vi "GLIMPSE Sequence Player.vi"() -> (8 "Sequence Range":cluster{i32, i32})   [LabVIEW 2015]
doc: "Allows the user to view and analyze a sequence of video stored as a temporary file on the disk. Also includes tools for setting areas of interest, manual tracking, automatic tracking by image fitting, etc."
uses:
  Header file data.ctl
  Seq file v 1/Offset table.ctl
  Seq file v 1/Offset.ctl
  Seq file v 1/file number.ctl
  Header2 file data.ctl
  <vilib>/vision/Image Controls.llb/IMAQ Image.ctl
  GLIMPSE Globals.vi
  <vilib>/Utility/file.llb/Write To Spreadsheet File (I64).vi
  AOI/AOI List Globals.vi
  <vilib>/Utility/NIReport.llb/NI_ReportGenerationCore.lvlib
panel:
  out "Header2 data":T1
  in  "Exit":bool
  out "Acquisition refnum array":refnum<file>[](array[refnum])
  out "file path":path
  out "Header data":T2 {"Pixel depth" items=["8 bits", "16 bits", "Float", "Complex", "RGB", "HSL"]; "time of 1st frame, \nsec since 1/1/04" format="%.2f"}
  in  "Change File":bool
  in  "Tab Control":T6(tab)
  in  "Overlay?":bool=TRUE caption="Loop?"
  in  "Frames to Step":u32=1 min=1 step=1
  in  "# Display\nWindows":i32=1 min=0 max=8 step=1
  in  "Delay between frames (msec)":i32=33 min=0 max=2147483600 step=100
  in  "Stop!":bool
  out "Time after 1st\nFrame (ms)":u32
  out "Mode":T7(ring)
  out "Time\nStamp":u32
  in  "Step Backward":bool
  in  "Step Forward":bool
  in  "Play Backward":bool
  in  "Play Forward":bool
  in  "Go to End":bool
  in  "Go to Begin":bool
  in  "Toggle beg/end":bool
  in  "Set end":bool
  in  "Set begin":bool
  in  "Loop?":bool=TRUE
  in  "Range Enabled":bool=TRUE caption="Restrict playback to range"
  in  "Frame Number":cluster{u32, u32}(slide)={10, 1} scale=1.0..13.0
  in  "Current Frame Number":u32(slide) max=13 scale=1.0..13.0
  out "Rev bkd":bool
  out "Fwd bkd":bool
  out "Stop bkgd":bool
  out "Filter":u16
  out "Field":u16
  out "Lasers":bool[](array[boolean])
  out "Flow":dbl
  out "Temp":dbl
  in  "Total FOVs":i16=4
  in  "Display FOV number":i16(slide)=1 min=1 scale=1.0..4.0
  in  "FOV Mode":T8(ring)=enum."Display all frames"
  in  "Printer":u16(ring) items=["Send To OneNote 16", "prism", "Microsoft XPS Document Writer", "Lab HP Color LaserJet M553", "Fax", "\\\\papercut\\Brandeis Ricoh Color", "\\\\papercut\\Brandeis Ricoh BW"]
  in  "Track by Curve Fitting to AOIs":bool
  in  "Print Image":bool
  in  "Save Portion of Current Frame":bool
  in  "Save Sequence":bool
  in  "Set/Modify AOIs (F8)":bool
  in  "Clear All":bool
  in  "Erase Last Row":bool
  out "Tracking Output File":path
  out "Number of Points":i16
  in  "Table":string[][](table)
  out "Pixel depth":u32(ring) items=["8 bits", "16 bits", "Float", "Complex", "RGB", "HSL"]
  out "Number of Frames":u32
  out "Frame width":i32
  out "Frame height":i32
  out "Camera":string
  out "Microscope":string
  out "Microscope software version":string
  out "Filter names":string[](array[string])
  out "Laser names":string[](array[string])
  # "These parameters are not for interactive use:"
  # "1"
  # "1"
  # "(F1)"
  # "(F2)"
  # "(F3)"
  # "(F4)"
  # "(F12)"
  # "Begin"
  # "Set"
  # "End"
  # "To add an (X, Y, T) point to table, click on image #1 with the point tool (\"+\")."
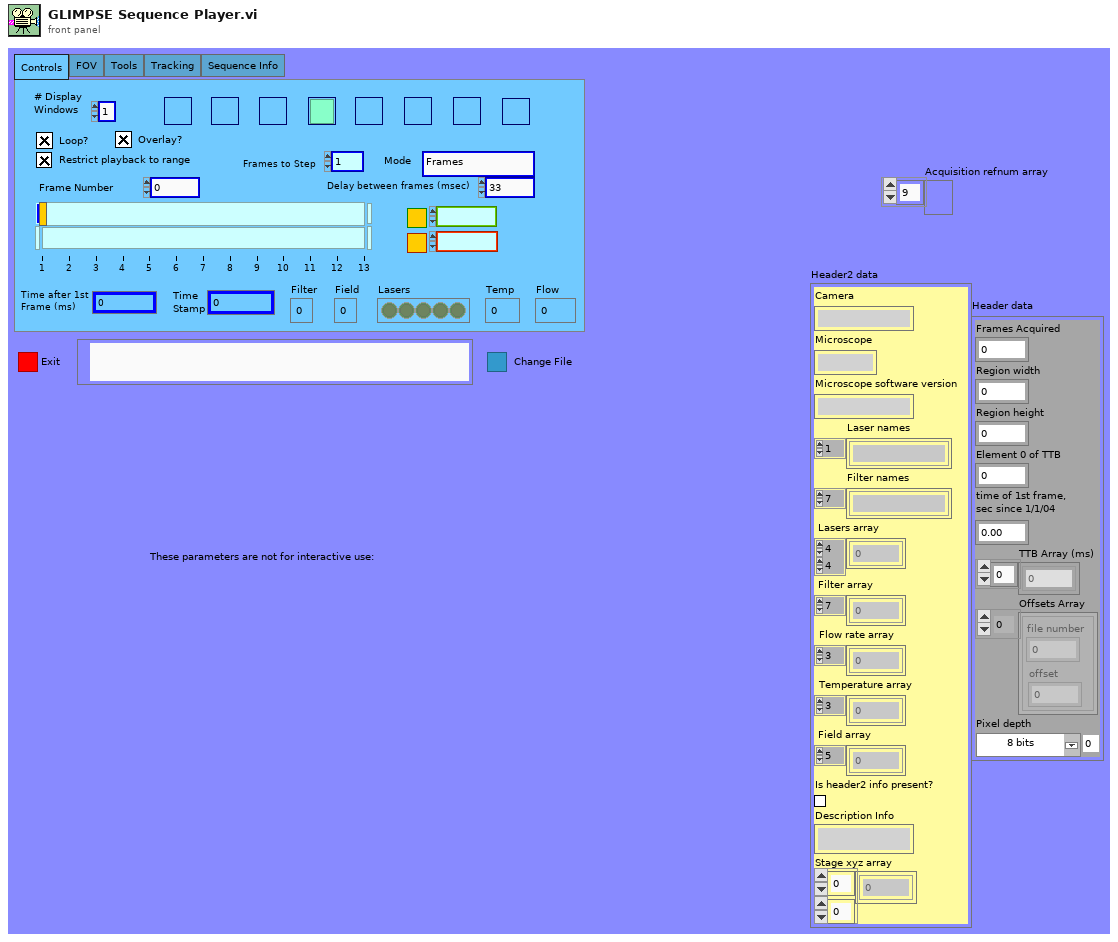
[diagram p1: front panel]
types:
  T1 = typedef "Header2 file data.ctl" = cluster{"Camera":string, "Microscope":string, "Microscope software version":string, "Laser names":string[], "Filter names":string[], "Lasers array":u16[][], "Filter array":u16[], "Flow rate array":dbl[], "Temperature array":dbl[], "Field array":u16[], "Is header2 info present?":bool, "Description Info":string, "Stage xyz array":dbl[][]}
  T2 = typedef "Header file data.ctl" = cluster{"Frames Acquired":u32, "Region width":i32, "Region height":i32, "Element 0 of TTB":u32, "time of 1st frame, \nsec since 1/1/04":dbl, "TTB Array (ms)":u32[], "Offsets Array":T3, "Pixel depth":u32}
  T3 = typedef "Offset table.ctl" = cluster{"offset":T4, "file number":T5}[]
  T4 = typedef "Offset.ctl" = i32
  T5 = typedef "file number.ctl" = u8
  T6 = enum32{"Controls", "FOV", "Tools", "Tracking", "Sequence Info"}
  T7 = enum16{"Frames", "Fields, Odd 1st", "Fields, Even 1st", "Fields, Averaged"}
  T8 = enum16{"Display one field of view", "Display all frames"}
  T9 = typedef "IMAQ Image.ctl" = refnum<image>
  T10 = enum32{"No Selection", "Point", "Line", "Rectangle", "Oval", "Polygon", "Free", "Unused1", "Zoom", "Unused2", "Broken Line", "Free Hand Line"}
  T11 = enum32{"No  event", "Click event", "Draw event", "Move event", "Size event", "Scroll event", "Activate event", "Close event", "Reserved"}[]
  T12 = cluster{"# of Frames Out (Log)":u32, "Current Frame Number":u32}
  T13 = cluster{"Left":i32, "Top":i32, "Right":i32, "Bottom":i32}
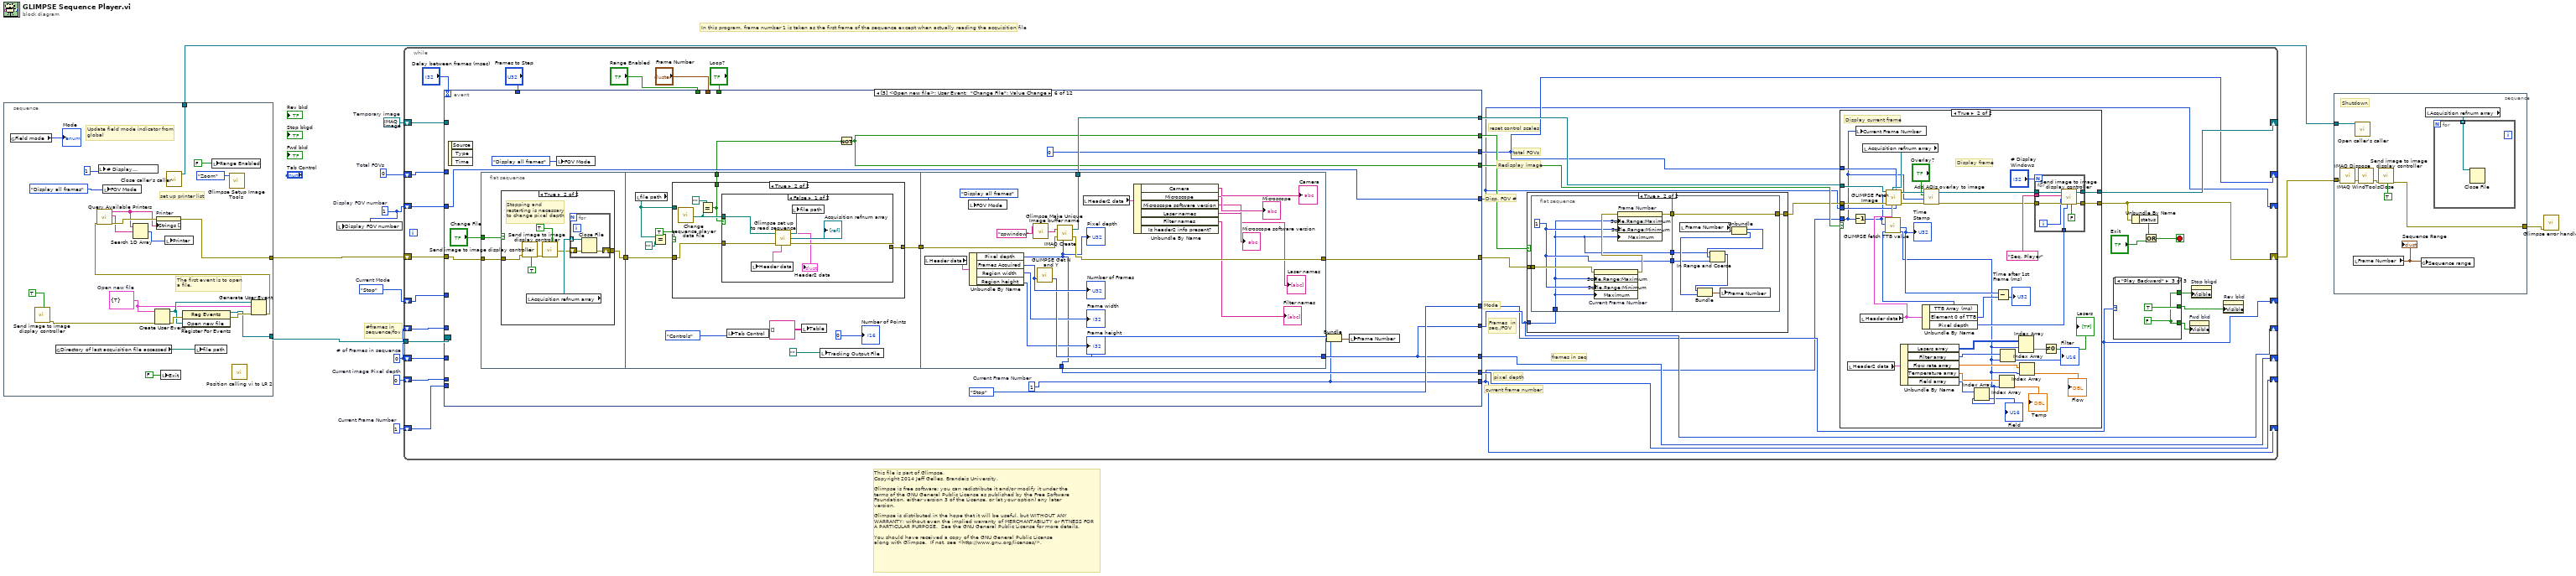
[diagram p0: block diagram]
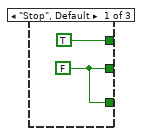
[diagram p2: hidden frame]
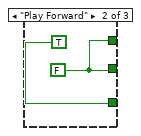
[diagram p3: hidden frame]
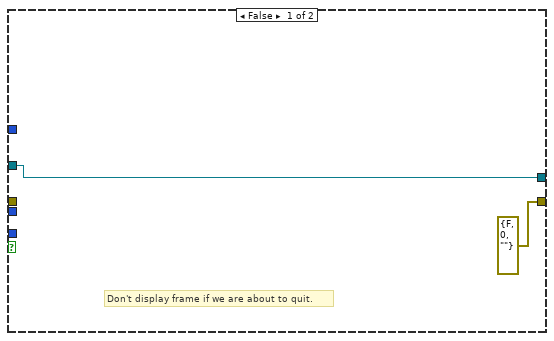
[diagram p4: hidden frame]
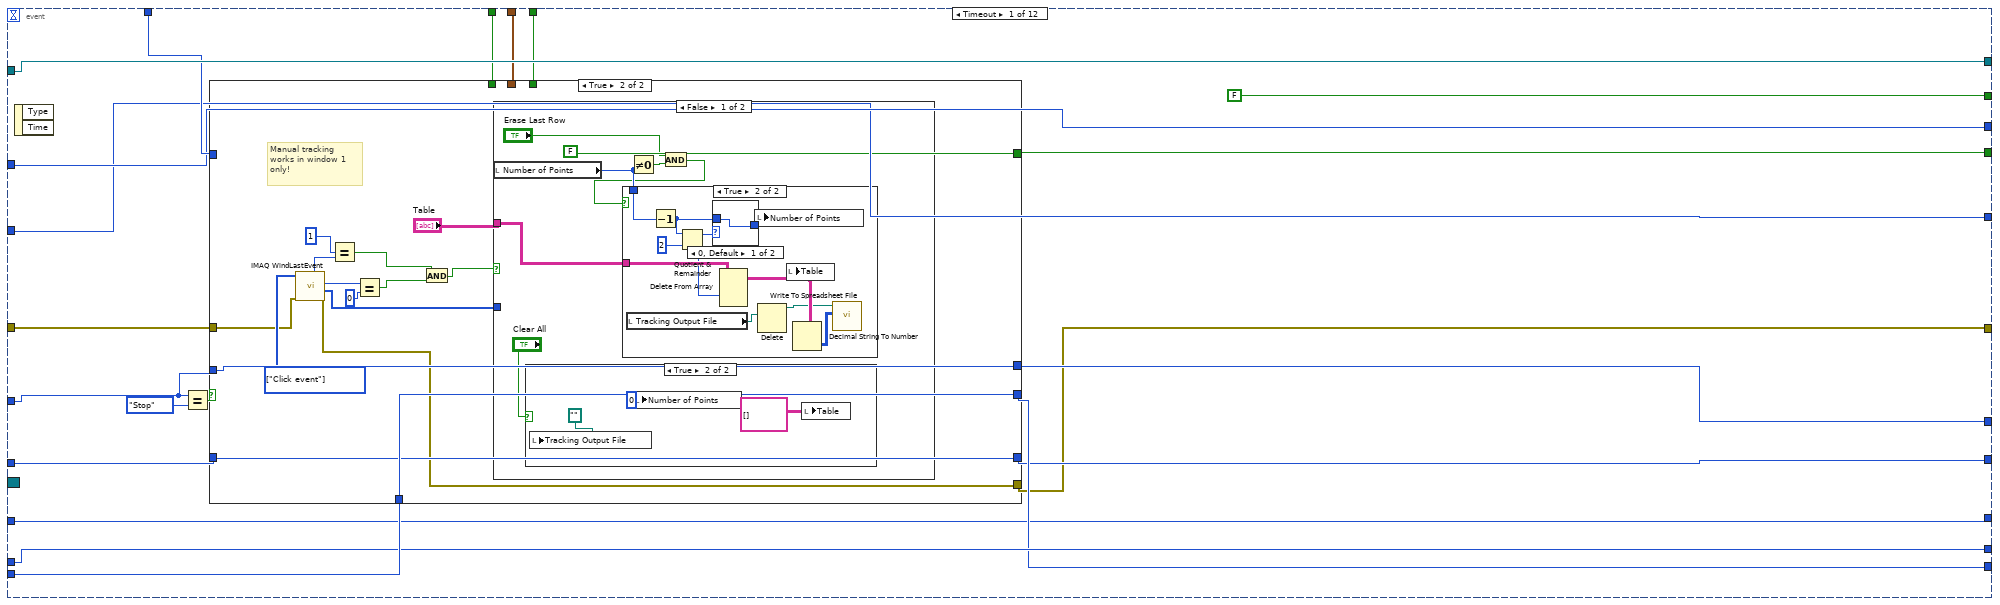
[diagram p6: hidden frame]
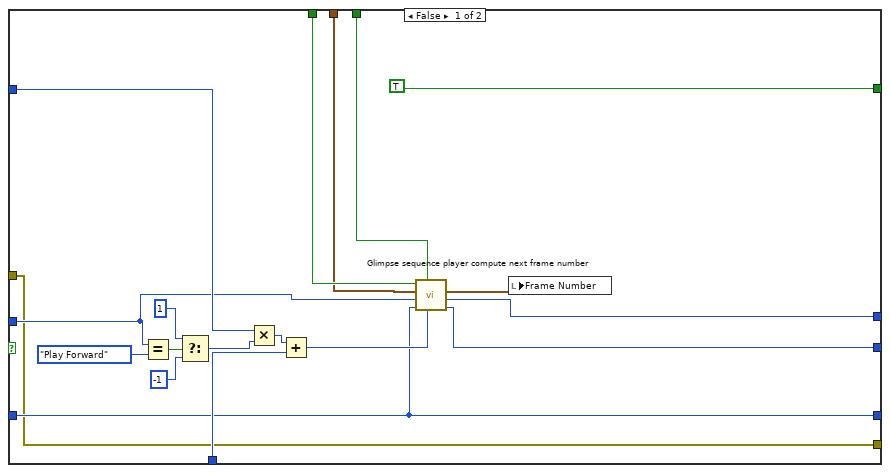
[diagram p7: hidden frame]
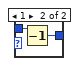
[diagram p10: hidden frame]
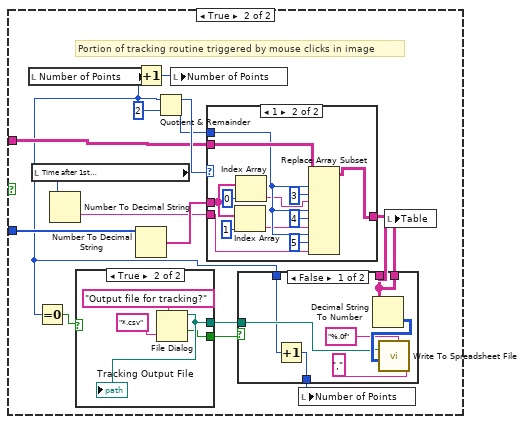
[diagram p11: hidden frame]
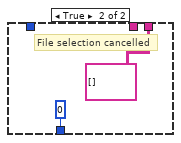
[diagram p12: hidden frame]
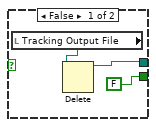
[diagram p13: hidden frame]
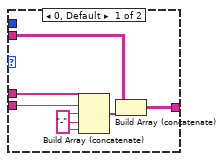
[diagram p14: hidden frame]
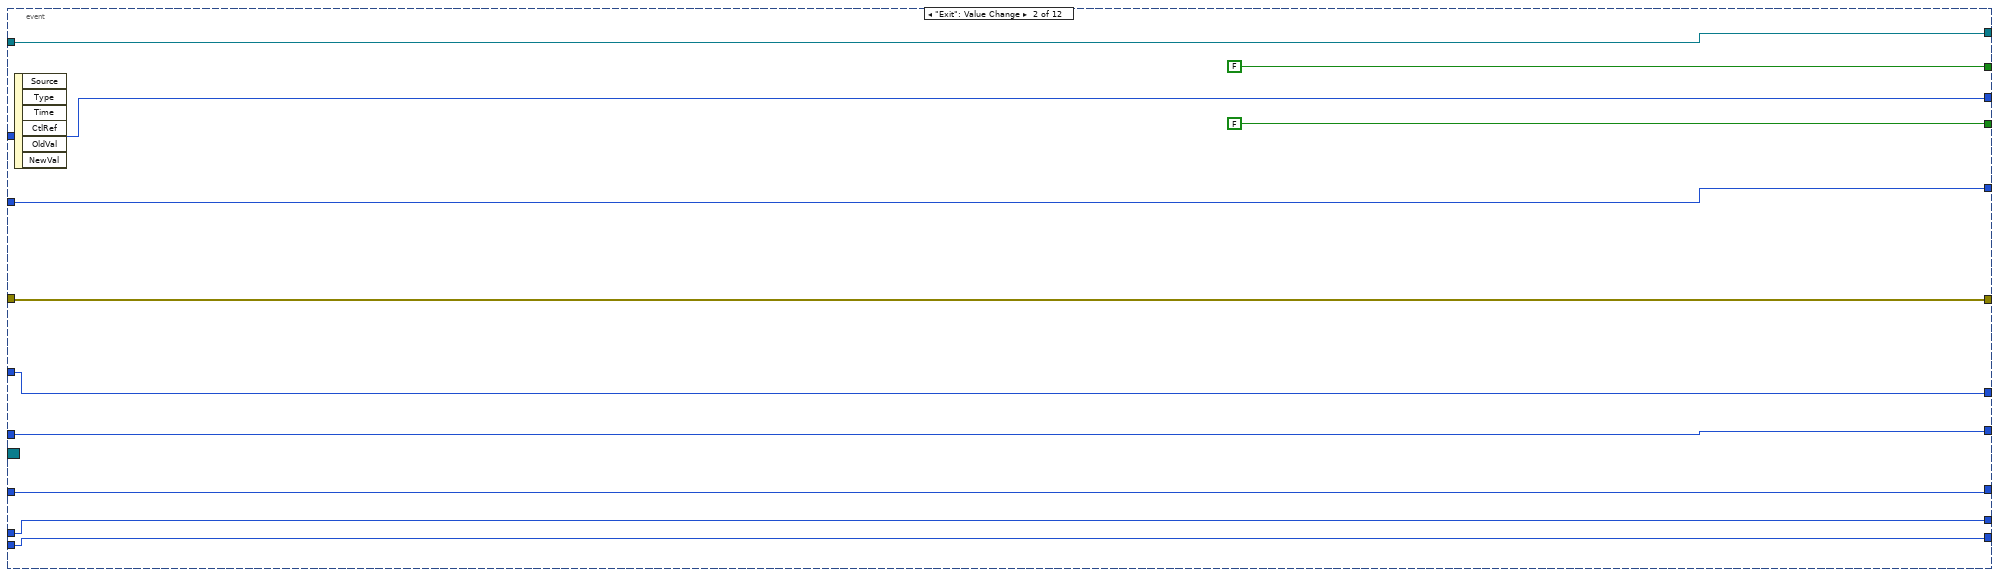
[diagram p15: hidden frame]
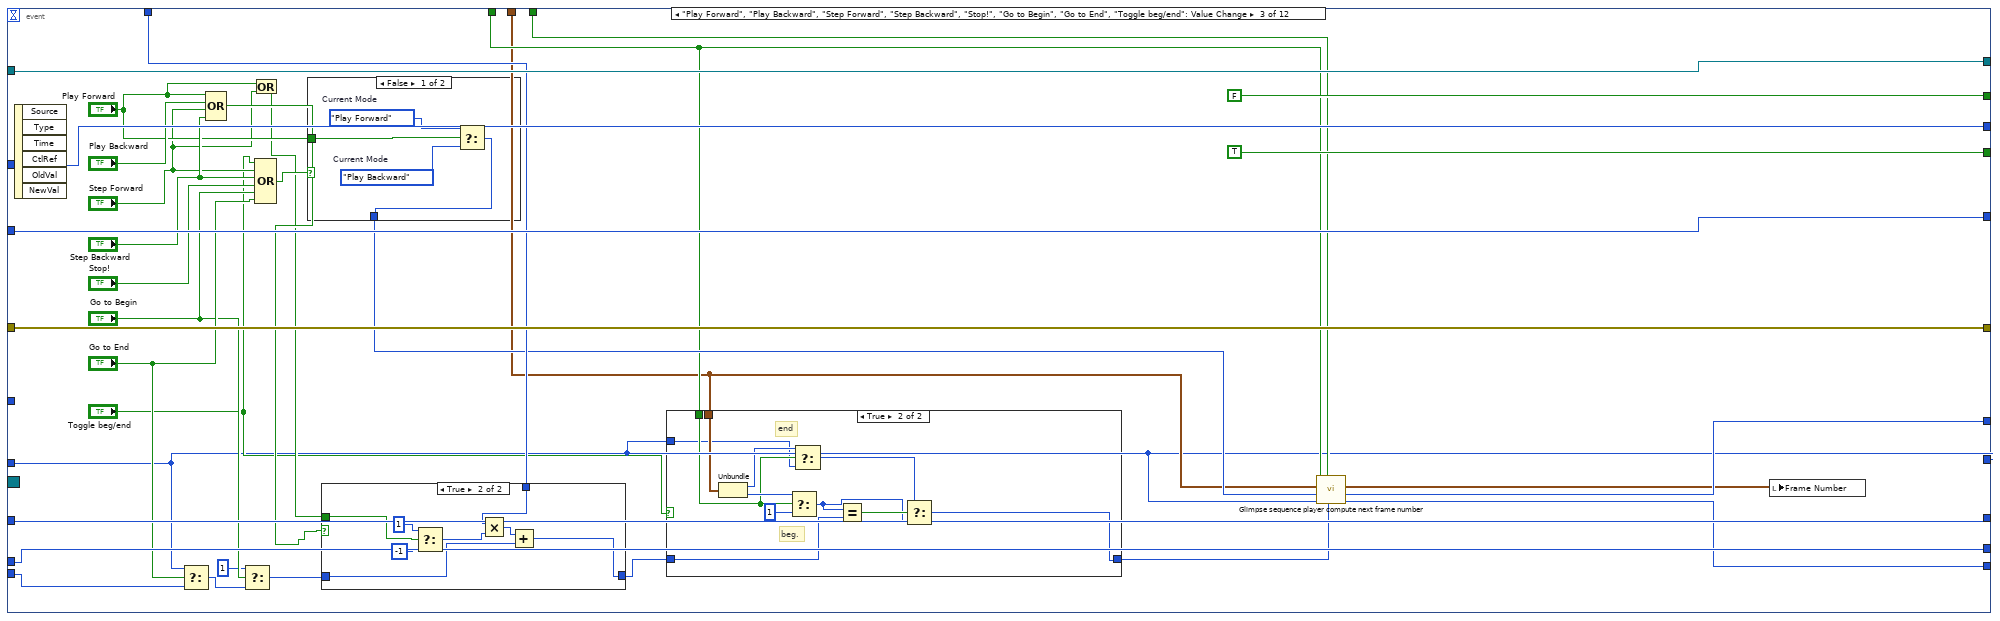
[diagram p16: hidden frame]
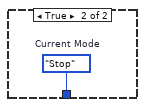
[diagram p19: hidden frame]
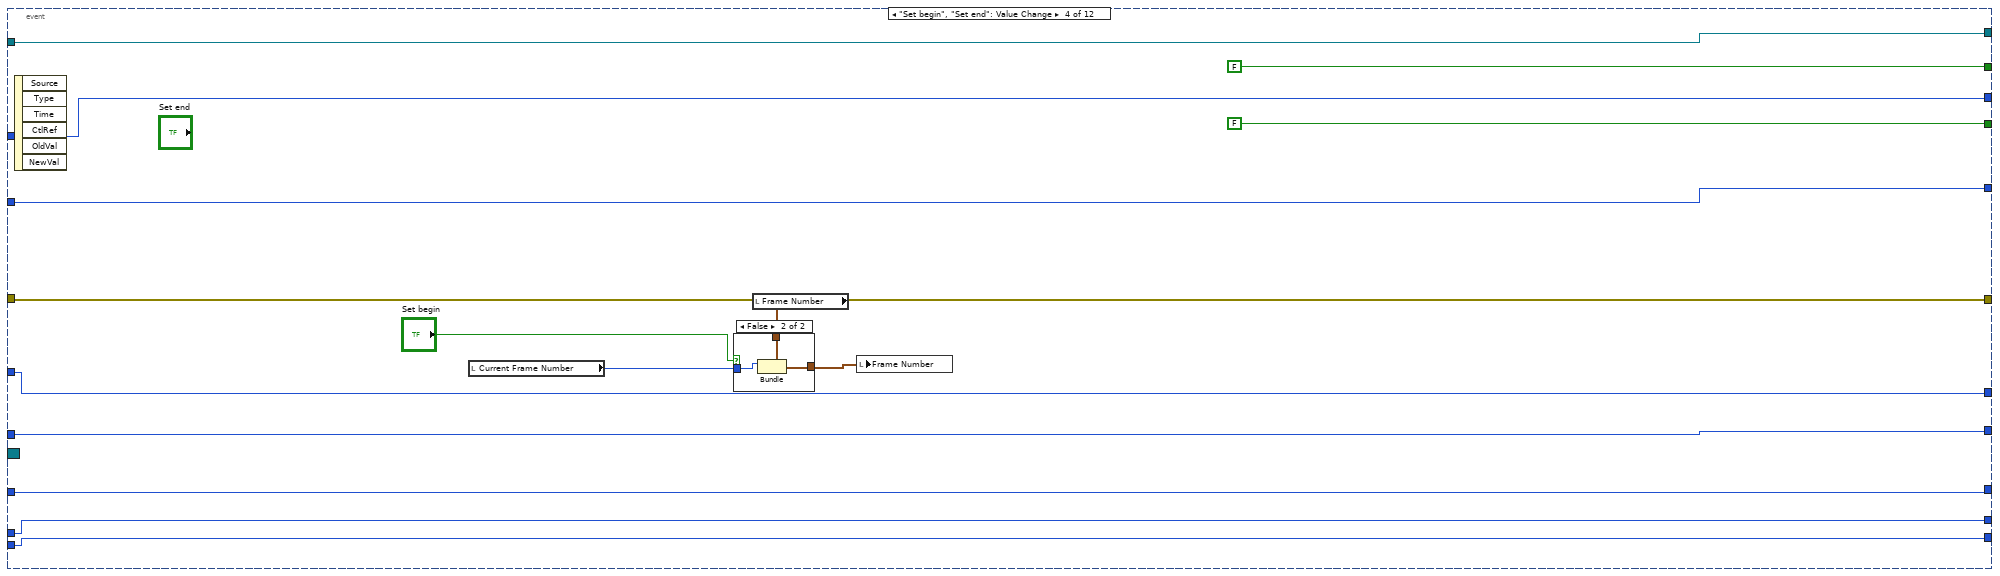
[diagram p20: hidden frame]
diagram:
  w3 = u32 0  # # of Frames in sequence
  w6 = T9 refnum  # Temporary image
  w4 = i16 1  # Display FOV number
  w7 = i16 0  # Total FOVs
  w8 = u32 0  # Current image Pixel depth
  w11 = u32 1  # Current Frame Number
  w5 = enum16{"Stop", "Play Forward", "Play Backward"}."Stop"  # Current Mode
  # "This file is part of Glimpse. \nCopyright 2014 Jeff Gelles, Brandeis University.    \n\nGlimpse is free software: you can redistribute it and/or modify it under the \nterms of the GNU General Public License as published by the Free Software \nFoundation, either version 3 of the License, or (at your option) any later \nversion.\n\nGlimpse is distributed in the hope that it will be useful, but WITHOUT ANY \nWARRANTY; without even the implied warranty of MERCHANTABILITY or FITNESS FOR \nA PARTICULAR PURPOSE.  See the GNU General Public License for more details.\n\nYou should have received a copy of the GNU General Public License\nalong with Glimpse.  If not, see <http://www.gnu.org/licenses/>."
  # "#frames in\nsequence/fov"
  # "In this program, frame number 1 is taken as the first frame of the sequence except when actually reading the acquisition file"
  n1 = stacked-sequence {
    tunnel: [w32] -> w12
    tunnel: [w21] -> w10
    tunnel: [w17] -> w9
    frame #0 {
      w14 = cluster{"dummy":bool} {"dummy"=TRUE}  # Open new file
      # "Update field mode indicator from\nglobal"
      # "The first event is to open\na file."
      # "set up printer list"
      n2 = global read "GLIMPSE Globals.vi" "Field mode"() -> (→"Mode":T7)
      n3 = call "Send image to image display controller.vi"("Start display controller?"=TRUE ("Quit display controller?")) -> ("error out"=w18:errorcluster)  [unwired: 6 in, 3 out]
      n4 = global read "GLIMPSE Globals.vi" "Directory of last acquisition file accessed"() -> (w25:path)
      n5 = local write "# Display\nWindows"(1 ("# Display\nWindows")) -> ()
      n6 = local write "FOV Mode"(T8."Display all frames" ("FOV Mode")) -> ()
      n7 = Create User Event(user event datatype=w14, error in=w18) -> (user event=w22:refnum<user-event>, error out=w24:errorcluster)
      n8 = local write "Exit"(FALSE ("Exit")) -> ()
      n9 = call "Close caller's caller.vi"() -> ("vi reference"=w32:refnum<vi>)  [unwired: 1 in, 7 out]
      n10 = register-events(error in=w24, w22) -> (reference out=w21:refnum<event-registration>, error out=w23:errorcluster)  [unwired: 1 in]
      n11 = local write "file path"(w25) -> ()
      n12 = local write "Range Enabled"(FALSE ("Exit")) -> ()
      n13 = call "Glimpse Setup Image Tools"("Default Tool"=T10."Zoom") -> ()  [unwired: 1 in, 3 out]
      n14 = call "Position calling vi to LR 2.vi"() -> ()  [unwired: 2 in, 4 out]
      n15 = Generate User Event(user event=w22, event data cluster=w14, error in=w23) -> (error out=w20:errorcluster)  [unwired: 1 in, 1 out]
      n16 = call <vilib>:"Query Available Printers.vi"("error in (no error)"=w20) -> ("error out"=w30:errorcluster, "default printer"=w29:string, "system configured printers"=w28:string[])  [unwired: 8 out]
      n17 = Search 1D Array(1D array=w28, element=w29) -> (index of element=w27:i32)  [unwired: 1 out]
      n18 = property on="Printer" class="Ring (strict)"(error in=w30, "Strings []"=w28) -> (error out=w17:errorcluster)  [unwired: 1 in, 1 out]
      n19 = local write "Printer"(w27) -> ()
    }
  }
  n20 = local write "Display FOV number"(w4) -> ()
  n21 = while {
    shift-right: [w34] -> _
    shift-left: w11 -> [w66]
    tunnel: w10 -> [w68]
    shift-right: [w43] -> w2
    shift-left: w9 -> [w67]
    shift-right: [w56] -> _
    shift-left: w6 -> [w61]
    shift-right: [w65] -> _
    shift-left: w8 -> [w64]
    shift-right: [w47] -> _
    shift-left: w7 -> [w63]
    shift-right: [w46] -> _
    shift-left: w4 -> [w62]
    shift-right: [w38] -> _
    shift-left: w5 -> [w60]
    shift-right: [w55] -> _
    shift-left: w3 -> [w59]
    shift-right: [w39] -> _
    shift-left: w3 -> [w45]
    stop <- w44 stop-if-true
    (unwired) cluster{string, u32}[] [] ("Images")
    # "pixel depth"
    # "frames in seq"
    # "Frames  in\nseq./FOV"
    # "Mode"
    # "Disp. FOV #"
    # "total FOVs"
    # "current frame number"
    # "Redisplay image"
    # "reset control scales"
    n22 = event shown="[5] <Open new file>: User Event;  \"Change File\": Value Change" {
      selector: w68 -> [_ _ _ _ _ _ _ _ _ _ _ _]
      dyn-events: _ -> [_ _ _ _ _ _ _ _ _ _ _ _]
      timeout: "Delay between frames (msec)" -> [_ _ _ _ _ _ _ _ _ _ _ _]
      tunnel: w67 -> [w141 w272 w309 w347 w366 w398 w504 w527 w551 w580 w594 w622]
      tunnel: [w158 w279 w313 w354 w372 w395 w466 w529 w550 w584 w595 w623] -> w57
      tunnel: [w140 w272 w309 w347 w366 w394 w473 w527 w538 w580 w593 w622] -> w49
      tunnel: [FALSE ("Reset control scales?") FALSE ("Reset control scales?") FALSE ("Reset control scales?") FALSE ("Reset control scales?") FALSE ("Reset control scales?") w383 w471 w531 w553 w586 TRUE ("Reset control scales?") w627] -> w58
      tunnel: w66 -> [w153 w278 w302 w353 w371 _ w463 w533 w548 w583 w601 _]
      tunnel: [w150 w278 w290 w353 w371 w386 w463 w533 w548 w583 w598 "Current Frame Number"] -> w34
      tunnel: [w151 w277 w312 w352 w370 w391 w474 w532 w547 w582 w599 w625] -> w65
      tunnel: w64 -> [w151 w277 w312 w352 w370 _ w474 w532 w547 w582 w599 w625]
      tunnel: w63 -> [w152 w269 w306 w344 w363 _ w469 w528 w543 w579 _ w618]
      tunnel: w62 -> [w143 w273 w310 w348 w367 w389 w468 w526 w540 w577 _ w619]
      tunnel: w61 -> [w158 w279 w313 w354 w372 _ w467 w529 w550 w584 w595 w623]
      tunnel: w60 -> [w155 w274 _ w349 _ _ _ _ w549 w578 w592 w621]
      tunnel: [w145 w274 w288 w349 w361 enum16{"Stop", "Play Forward", "Play Backward"}."Stop" ("Current Mode") enum16{"Stop", "Play Forward", "Play Backward"}."Stop" ("Current Mode") enum16{"Stop", "Play Forward", "Play Backward"}."Stop" ("Current Mode") w549 w578 w592 w621] -> w38
      tunnel: [w144 w276 w311 w351 w369 w387 w464 w524 w546 w581 w597 w624] -> w55
      tunnel: w59 -> [w144 w276 w311 w351 w369 _ w464 w524 w546 w581 w597 w624]
      tunnel: [w152 w269 w306 w344 w363 i16 0 ("Total FOVs") w469 w528 w543 w579 w605 w618] -> w47
      tunnel: [w143 w273 w310 w348 w367 w389 w468 w526 w540 w577 w604 w619] -> w46
      tunnel: [w142 w275 w280 w350 w368 w387 w465 w525 w545 w576 w602 w620] -> w39
      tunnel: [w156 FALSE ("Redisplay image") TRUE ("Redisplay image") FALSE ("Redisplay image") FALSE ("Redisplay image") w383 w470 w530 w552 w585 TRUE ("Redisplay image") w626] -> w50
      tunnel: w45 -> [w149 w275 w280 w350 w368 _ w465 w525 w545 w576 _ w620]
      tunnel: "Frames to Step" -> [w154 _ w294 _ _ _ _ _ _ _ _ _]
      tunnel: "Loop?" -> [w148 _ w287 _ _ _ _ _ _ _ _ _]
      tunnel: "Range Enabled" -> [w147 _ w282 _ _ _ _ _ _ _ _ _]
      tunnel: "Frame Number" -> [w146 _ w281 _ w362 _ _ _ _ _ _ _]
      event Timeout {
        n23 = event-data() -> ()  [unwired: 3 out]
        n24 = Equal?(x=w155, y=enum16{"Stop", "Play Forward", "Play Backward"}."Stop") -> (x = y?=w160:bool)
        n25 = case shown="True" w160 {
          tunnel: [TRUE ("Reset control scales?") FALSE ("Reset control scales?")] -> w156
          tunnel: w155 -> [w166 w193]
          tunnel: w154 -> [w176 _]
          tunnel: w153 -> [w171 w194]
          tunnel: [w164 w194] -> w150
          tunnel: w149 -> [w162 w192]
          tunnel: w148 -> [w169 _]
          tunnel: w147 -> [w168 _]
          tunnel: w146 -> [w167 _]
          tunnel: [w163 w193] -> w145
          tunnel: [w162 w192] -> w142
          tunnel: w141 -> [w161 w181]
          tunnel: [w161 w180] -> w140
          frame False {
            n26 = Equal?(x=w166, y=enum16{"Stop", "Play Forward", "Play Backward"}."Play Forward") -> (x = y?=w177:bool)
            n27 = Select(t=1, s=w177, f=-1) -> (s? t:f=w175:i32)
            n28 = Multiply(x=w176, y=w175) -> (x*y=w172:u32)
            n29 = Add(x=w172, y=w171) -> (x+y=w165:u32)
            n30 = call "Glimpse sequence player compute next frame number.vi"("Current Frame Number"=w165, "Loop?"=w169, "# of Frames in sequence/FOV"=w162, "Current Mode"=w166, "Range In"=w167, "Range Enabled"=w168) -> ("Current Frame Number Out"=w164:u32, "Current Mode Out"=w163:enum16{"Stop", "Play Forward", "Play Backward"}, "Range Out"=w170:cluster{"Max":u32, "Min":u32})  [unwired: 1 out]
            n31 = local write "Frame Number"(w170) -> ()
          }
          frame True {
            w190 = T11 [enum."Click event"] items=["No  event", "Click event", "Draw event", "Move event", "Size event", "Scroll event", "Activate event", "Close event", "Reserved"] ("Events list (all)")
            # "Manual tracking \nworks in window 1\nonly!"
            n32 = call "IMAQ WindLastEvent"("error in (no error)"=w181, "Events list (all)"=w190) -> ("error out"=w180:errorcluster, "Coordinates"=w184:i32[], "Tool"=w189:i32, "Window Number (0...15)"=w191:i32)  [unwired: 6 out]
            n33 = Equal?(x=1 ("Window Number (0...15)"), y=w191) -> (x = y?=w186:bool)
            n34 = Equal?(x=w189, y=0) -> (x = y?=w187:bool)
            n35 = And(x=w186, y=w187) -> (x .and. y?=w185:bool)
            n36 = case shown="False" w185 {
              tunnel: w184 -> [_ w230]
              tunnel: "Table" -> [w200 w224]
              frame False {
                n37 = local read "Number of Points"() -> (w199:i16)
                n38 = case shown="True" "Clear All" {
                  frame False {
                  }
                  frame True {
                    n39 = local write "Tracking Output File"(path "") -> ()
                    n40 = local write "Number of Points"(i16 0 ("Number of Points")) -> ()
                    n41 = local write "Table"(string[][] []) -> ()
                  }
                }
                n42 = Not Equal To 0?(x=w199) -> (x != 0?=w198:bool)
                n43 = And(x="Erase Last Row", y=w198) -> (x .and. y?=w197:bool)
                n44 = case shown="True" w197 {
                  tunnel: w200 -> [_ w211]
                  tunnel: w199 -> [_ w206]
                  frame False {
                  }
                  frame True {
                    n45 = local read "Tracking Output File"() -> (w205:path)
                    n46 = Decrement(x=w206) -> (x-1=w214:i16)
                    n47 = Quotient & Remainder(x=w214, y=i16 2) -> (x-y*floor(x/y)=w212:i16, floor(x/y)=w210:i16)
                    n48 = case shown="0, Default" w212 {
                      tunnel: w214 -> [w216 w218]
                      tunnel: [w216 w217] -> w213
                      frame 0, Default {
                      }
                      frame 1 {
                        n49 = Decrement(x=w218) -> (x-1=w217:i16)
                      }
                    }
                    n50 = Delete From Array(array=w211, index (row)=w210) -> (array with subset deleted=w209:string[][])  [unwired: 2 in, 1 out]
                    n51 = local write "Number of Points"(w213) -> ()
                    n52 = Delete(path (use dialog)=w205) -> (deleted path=w208:path)  [unwired: 1 in, 5 out]
                    n53 = local write "Table"(w209) -> ()
                    n54 = Decimal String To Number(string=w209) -> (number=w207:i32[][])  [unwired: 3 out]
                    n55 = call-poly <vilib>:"Write To Spreadsheet File.vi"("2D data"=w207, "file path (dialog if empty)"=w208) -> ()  [unwired: 4 in, 3 out]
                  }
                }
              }
              frame True {
                # "Portion of tracking routine triggered by mouse clicks in image"
                n56 = local read "Number of Points"() -> (w221:i16)
                n57 = local read "Time after 1st\nFrame (ms)"() -> (w231:u32)
                n58 = Equal To 0?(x=w221) -> (x = 0?=w226:bool)
                n59 = Number To Decimal String(number=w231) -> (decimal integer string=w228:string)  [unwired: 1 out]
                n60 = case shown="True" w226 {
                  tunnel: [w245 w248] -> w222
                  tunnel: [FALSE ("cancelled") w247] -> w223
                  frame False {
                    n61 = local read "Tracking Output File"() -> (w246:path)
                    n62 = Delete(path (use dialog)=w246) -> (deleted path=w245:path)  [unwired: 1 in, 5 out]
                  }
                  frame True {
                    n63 = File Dialog(6:"*.csv" ("pattern"), 7:"Output file for tracking?" ("prompt")) -> (1:w247:bool, 3:w248:path)  [unwired: 1 in, 6 out]
                    "Tracking Output File" <- w248
                  }
                }
                n64 = Increment(x=w221) -> (x+1=w233:i16)
                n65 = Number To Decimal String(number=w230) -> (decimal integer string=w229:string[])  [unwired: 1 in]
                n66 = Quotient & Remainder(x=w221, y=i16 2) -> (x-y*floor(x/y)=w232:i16, floor(x/y)=w227:i16)
                n67 = local write "Number of Points"(w233) -> ()
                n68 = case shown="1" w232 {
                  tunnel: w224 -> [w256 w268]
                  tunnel: [w253 w267] -> w225
                  tunnel: w229 -> [w252 w261]
                  tunnel: w228 -> [w251 w262]
                  tunnel: w227 -> [_ w263]
                  frame 0, Default {
                    w254 = "-"
                    n69 = Build Array (concatenate)(w252, w251, w254, w254, w254) -> (w255:string[])
                    n70 = Build Array (concatenate)(w256, w255) -> (w253:string[][])
                  }
                  frame 1 {
                    n71 = Index Array(array=w261, index=1 ("Index")) -> (element=w257:string)
                    n72 = Index Array(array=w261, index=0 ("Index")) -> (element=w258:string)
                    n73 = Replace Array Subset(array=w268, new element #1=w258, index (row) #1=w263, index (col) #1=3 ("Disabled Index (col)"), new element #2=w257, index (row) #2=w263, index (col) #2=4 ("Index (col)"), new element #3=w262, index (row) #3=w263, index (col) #3=5 ("Index (col)")) -> (w267:string[][])
                  }
                }
                n74 = case shown="False" w223 {
                  tunnel: w225 -> [w237 _]
                  tunnel: w222 -> [w240 _]
                  tunnel: w221 -> [w239 _]
                  tunnel: [w238 i16 0] -> w220
                  tunnel: [w237 string[][] []] -> w219
                  frame False {
                    n75 = Increment(x=w239) -> (x+1=w238:i16)
                    n76 = Decimal String To Number(string=w237) -> (number=w241:i32[][])  [unwired: 3 out]
                    n77 = call-poly <vilib>:"Write To Spreadsheet File.vi"("delimiter (\\t)"="," ("delimiter (Tab)"), "format (%d)"="%.0f" ("format (%.3f)"), "2D data"=w241, "file path (dialog if empty)"=w240) -> ()  [unwired: 3 in, 2 out]
                  }
                  frame True {
                    # "File selection cancelled"
                  }
                }
                n78 = local write "Number of Points"(w220) -> ()
                n79 = local write "Table"(w219) -> ()
              }
            }
          }
        }
      }
      event "Exit": Value Change {
        n80 = event-data() -> ()  [unwired: 7 out]
      }
      event "Play Forward", "Play Backward", "Step Forward", "Step Backward", "Stop!", "Go to Begin", "Go to End", "Toggle beg/end": Value Change {
        n81 = event-data() -> ()  [unwired: 7 out]
        n82 = Select(t=w280, s="Go to End", f=w302) -> (s? t:f=w300:u32)
        n83 = Compound Arithmetic op=OR("Play Forward", "Play Backward", "Step Forward", "Step Backward") -> (w296:bool)
        n84 = Select(t=u32 1, s="Go to Begin", f=w300) -> (s? t:f=w295:u32)
        n85 = Or(x="Play Forward", y="Step Forward") -> (x .or. y?=w291:bool)
        n86 = Compound Arithmetic op=OR("Toggle beg/end", "Step Forward", "Step Backward", "Stop!", "Go to Begin", "Go to End") -> (w304:bool)
        n87 = case shown="False" w304 {
          tunnel: [w335 w339] -> w289
          tunnel: "Play Forward" -> [w338 _]
          frame False {
            w336 = enum16{"Stop", "Play Forward", "Play Backward"}."Play Backward"  # Current Mode
            w337 = enum16{"Stop", "Play Forward", "Play Backward"}."Play Forward"  # Current Mode
            n88 = Select(t=w337, s=w338, f=w336) -> (s? t:f=w335:enum16{"Stop", "Play Forward", "Play Backward"})
          }
          frame True {
            w339 = enum16{"Stop", "Play Forward", "Play Backward"}."Stop"  # Current Mode
          }
        }
        n89 = case shown="True" w296 {
          tunnel: w295 -> [w326 w329]
          tunnel: [w326 w328] -> w284
          tunnel: w294 -> [_ w330]
          tunnel: w291 -> [_ w327]
          frame False {
          }
          frame True {
            n90 = Select(t=1, s=w327, f=-1) -> (s? t:f=w332:i32)
            n91 = Multiply(x=w330, y=w332) -> (x*y=w334:u32)
            n92 = Add(x=w334, y=w329) -> (x+y=w328:u32)
          }
        }
        n93 = case shown="True" "Toggle beg/end" {
          tunnel: w284 -> [w314 w324]
          tunnel: [w314 w315] -> w283
          tunnel: w282 -> [_ w319]
          tunnel: w281 -> [_ w322]
          tunnel: w280 -> [_ w317]
          frame False {
          }
          frame True {
            # "end"
            # "beg."
            n94 = Unbundle(w322) -> (w318:u32, w321:u32)
            n95 = Select(t=w321, s=w319, f=u32 1) -> (s? t:f=w320:u32)
            n96 = Select(t=w318, s=w319, f=w317) -> (s? t:f=w316:u32)
            n97 = Equal?(x=w320, y=w324) -> (x = y?=w323:bool)
            n98 = Select(t=w316, s=w323, f=w320) -> (s? t:f=w315:u32)
          }
        }
        n99 = call "Glimpse sequence player compute next frame number.vi"("Current Frame Number"=w283, "Loop?"=w287, "# of Frames in sequence/FOV"=w280, "Current Mode"=w289, "Range In"=w281, "Range Enabled"=w282) -> ("Current Frame Number Out"=w290:u32, "Current Mode Out"=w288:enum16{"Stop", "Play Forward", "Play Backward"}, "Range Out"=w286:cluster{"Max":u32, "Min":u32})  [unwired: 1 out]
        n100 = local write "Frame Number"(w286) -> ()
      }
      event "Set begin", "Set end": Value Change {
        n101 = event-data() -> ()  [unwired: 7 out]
        n102 = local read "Current Frame Number"() -> (w342:u32)
        n103 = local read "Frame Number"() -> (w341:cluster{u32, u32})
        n104 = case shown="False" "Set begin" {
          tunnel: [w357 w360] -> w343
          tunnel: w342 -> [w356 w358]
          tunnel: w341 -> [w355 w359]
          frame True {
            n105 = Bundle(cluster=w355, w356) -> (w357:cluster{u32, u32})  [unwired: 1 out]
          }
          frame False {
            n106 = Bundle(cluster=w359, w358) -> (w360:cluster{u32, u32})  [unwired: 1 out]
          }
        }
        n107 = local write "Frame Number"(w343) -> ()
      }
      event "Track by Curve Fitting to AOIs": Value Change {
        n108 = event-data() -> ()  [unwired: 7 out]
        n109 = flat-sequence {
          tunnel: [enum16{"Stop", "Play Forward", "Play Backward"}."Stop" ("Current Mode")] -> w361
          tunnel: w362 -> [w373]
          frame #0 {
            n110 = global read "GLIMPSE Globals.vi" "Current window Black/White Levels"() -> (w374:cluster{ext, ext})
            n111 = local read "Acquisition refnum array"() -> (w380:refnum<file>[])
            n112 = local read "Header data"() -> (w375:T2)
            n113 = Unbundle(w373) -> (w379:u32, w378:u32)
            n114 = Unbundle(w374) -> (w377:ext, w376:ext)
            n115 = call "fit aois.vi"("End frame"=w379, "White level"=w376, "Header Info"=w375, "Start frame"=w378, "Black level"=w377, "Acquisition refnum array"=w380) -> ()  [unwired: 5 out]
          }
          frame #1 {
            n116 = call "IMAQ WindToolsShow"() -> ("error out"=w382:errorcluster)  [unwired: 3 in, 3 out]
            n117 = call <vilib>:"Simple Error Handler.vi"("error in (no error)"=w382) -> ()  [unwired: 1 in, 8 out]
          }
        }
      }
      event User Event; "Change File": Value Change {
        w386 = u32 1  # Current Frame Number
        n118 = event-data() -> ()  [unwired: 4 out]
        n119 = flat-sequence {
          tunnel: w398 -> [w401]
          tunnel: [w400] -> w397
          tunnel: "Change File" -> [w399]
          tunnel: w397 -> [w420]
          tunnel: [w415] -> w396
          tunnel: [w413] -> w384
          tunnel: w396 -> [w459]
          tunnel: [w458] -> w395
          tunnel: [w457] -> w394
          tunnel: [w451] -> w391
          tunnel: [w455] -> w387
          frame #0 {
            n120 = case shown="True" w399 {
              tunnel: w401 -> [w402 w407]
              tunnel: [w402 w406] -> w400
              frame False {
              }
              frame True {
                # "Stopping and \nrestarting is necessary\nto change pixel depth"
                n121 = call "Send image to image display controller.vi"("error in"=w407, "Quit display controller?"=TRUE) -> ("error out"=w403:errorcluster)  [unwired: 5 in, 3 out]
                n122 = local read "Acquisition refnum array"() -> (w409:refnum<file>[])
                n123 = call "Send image to image display controller.vi"("error in"=w403, "Start display controller?"=TRUE ("Quit display controller?")) -> ("error out"=w408:errorcluster)  [unwired: 5 in, 3 out]
                n124 = for {
                  tunnel: w409 -> [w412] mode=indexing
                  shift-right: [w410] -> w406
                  shift-left: w408 -> [w411]
                  n125 = Close File(refnum=w412, error in=w411) -> (error out=w410:errorcluster)  [unwired: 1 out]
                }
              }
            }
          }
          frame #1 {
            n126 = local read "file path"() -> (w422:path)
            n127 = Equal?(x=w422, y=path "") -> ()  [unwired: 1 out]
            n128 = case shown="True" TRUE {
              tunnel: w422 -> [w430 _]
              tunnel: w420 -> [w426 w433]
              tunnel: [w425 w432] -> w415
              tunnel: [FALSE w431] -> w413
              frame False {
                # "automatically open last file accessed"
                n129 = call "Glimpse set up to read sequence.vi"("acquisition directory path"=w430, "error in"=w426) -> ("Header2 file data out"=w423:T1, "Header file data out"=→"Header data":T2, "acquisition directory path out"=→"file path":path, "Acquisition refnum array"=w428:refnum<file>[], "error out"=w425:errorcluster)  [unwired: 1 out]
                n130 = local write "Acquisition refnum array"(w428) -> ()
                n131 = local write "Header2 data"(w423) -> ()
              }
              frame True {
                n132 = call "Change sequence player data file.vi"() -> ("File path out"=w435:path)  [unwired: 1 in, 4 out]
                n133 = Equal?(x=path "", y=w435) -> (x = y?=w431:bool)
                n134 = case shown="False" w431 {
                  tunnel: w435 -> [w442 _]
                  tunnel: w433 -> [w438 w444]
                  tunnel: [w437 w444] -> w432
                  frame False {
                    n135 = call "Glimpse set up to read sequence.vi"("acquisition directory path"=w442, "error in"=w438) -> ("Header2 file data out"=→"Header2 data":T1, "Header file data out"=w439:T2, "acquisition directory path out"=w441:path, "Acquisition refnum array"=→"Acquisition refnum array":refnum<file>[], "error out"=w437:errorcluster)  [unwired: 1 out]
                    n136 = local write "Header data"(w439) -> ()
                    n137 = local write "file path"(w441) -> ()
                  }
                  frame True {
                    n138 = local write "Exit"(TRUE ("Exit")) -> ()
                  }
                }
              }
            }
            n139 = local write "Tab Control"(enum32{"Controls", "FOV", "Tools", "Tracking"}."Controls" ("Tab Control")) -> ()
            n140 = local write "Table"(string[][] []) -> ()
            n141 = local write "Tracking Output File"(path "") -> ()
            "Number of Points" <- i16 0 ("Number of Points")
          }
          frame #2 {
            n142 = local read "Header data"() -> (w462:T2)
            n143 = local write "FOV Mode"(T8."Display all frames" ("FOV Mode")) -> ()
            n144 = Unbundle By Name(w462) -> ("Pixel depth"=w451:u32, "Frames Acquired"=w456:u32, "Region width"=→"Frame width":i32, "Region height"=→"Frame height":i32)
            "Number of Frames" <- w456
            "Pixel depth" <- w451
            n145 = call "Glimpse Make Unique Image buffer name.vi"("Buffer  base name"="spwindow" ("Image Name")) -> ("Image Name"=w461:string)  [unwired: 1 out]
            n146 = call "GLIMPSE Get N and Y.vi"("# of Frames In (Phys)"=w456) -> ("# of Frames Out (Log)"=w455:u32)  [unwired: 2 in, 4 out]
            n147 = call "IMAQ Create"("Image Name"=w461, "Image Type"=w451, "error in (no error)"=w459) -> ("New Image"=w458:T9, "error out"=w457:errorcluster)  [unwired: 1 in, 1 out]
            n148 = local read "Header2 data"() -> (w450:T1)
            n149 = Unbundle By Name(w450) -> ("Camera"=→"Camera":string, "Microscope"=→"Microscope":string, "Microscope software version"=→"Microscope software version":string, "Laser names"=→"Laser names":string[], "Filter names"=→"Filter names":string[])  [unwired: 1 out]
          }
        }
        n150 = local write "FOV Mode"(T8."Display all frames" ("FOV Mode")) -> ()
        n151 = Not(x=w384) -> (.not. x?=w383:bool)
        n152 = Bundle("# of Frames Out (Log)"=w387, "Current Frame Number"=w386) -> (w388:T12)  [unwired: 1 out]
        n153 = local write "Frame Number"(w388) -> ()
      }
      event "Set/Modify AOIs (F8)": Value Change {
        w470 = TRUE  # Redisplay image
        w471 = FALSE  # Reset control scales?
        n154 = event-data() -> ()  [unwired: 7 out]
        n155 = call "IMAQ Create"("Image Name"="Field1", "Image Type"=w474, "error in (no error)"=w504) -> ("New Image"=w508:T9, "error out"=w501:errorcluster)  [unwired: 1 in, 1 out]
        n156 = call "IMAQ Create"("Image Name"="Field2", "Image Type"=w474, "error in (no error)"=w501) -> ("New Image"=w507:T9, "error out"=w480:errorcluster)  [unwired: 1 in, 1 out]
        n157 = local read "Header data"() -> (w481:T2)
        n158 = local read "Frame Number"() -> (w498:cluster{u32, u32})
        n159 = global read "GLIMPSE Globals.vi" "Current window Black/White Levels"() -> (w492:cluster{ext, ext})
        n160 = Unbundle(w498) -> (w500:u32, w499:u32)
        n161 = Decrement(x=w500) -> (x-1=w497:u32)
        n162 = Decrement(x=w499) -> (x-1=w496:u32)
        n163 = local read "Acquisition refnum array"() -> (w495:refnum<file>[])
        n164 = call "GLIMPSE Fetch Image.vi"("Display FOV number"=w468, "Total FOVs"=w469, "Header file data"=w481, "Acqisition files refnums"=w495, "error in"=w480, "Logical Frame Number\n(starting with zero)"=w497, "Image In"=w508) -> ("error out"=w479:errorcluster, "Image Out"=w506:T9)  [unwired: 3 out]
        n165 = call "GLIMPSE Fetch Image.vi"("Display FOV number"=w468, "Total FOVs"=w469, "Header file data"=w481, "Acqisition files refnums"=w495, "error in"=w479, "Logical Frame Number\n(starting with zero)"=w496, "Image In"=w507) -> ("error out"=w478:errorcluster, "Image Out"=w505:T9)  [unwired: 3 out]
        n166 = Unbundle(w492) -> (w494:ext, w493:ext)
        n167 = call "Multiple AOIs.vi"("White level"=w493, "Black level"=w494, "First (or only) image (red)"=w506, "error in"=w478, "Second image (green)"=w505, "Image Type"=w474) -> ("error out"=w477:errorcluster)  [unwired: 5 out]
        n168 = call "IMAQ WindToolsShow"("error in (no error)"=w477) -> ("error out"=w490:errorcluster)  [unwired: 2 in, 3 out]
        n169 = local write "Tab Control"(enum32{"Controls", "FOV", "Tools", "Tracking"}."Controls" ("Tab Control")) -> ()
        n170 = call "IMAQ Dispose"("Image"=w506, "error in (no error)"=w490) -> ("error out"=w491:errorcluster)  [unwired: 1 in, 3 out]
        n171 = call "IMAQ Dispose"("Image"=w505, "error in (no error)"=w491) -> ("error out"=w476:errorcluster)  [unwired: 1 in, 3 out]
        n172 = Open VI Reference(vi path=path "GLIMPSE Sequence Player.vi", error in (no error)=w476) -> (vi reference=w487:refnum<vi>, error out=w486:errorcluster)  [unwired: 4 out]
        n173 = property class="VI"(reference=w487, error in=w486, "Front Panel Window:Is Frontmost"=TRUE) -> (reference out=w483:refnum<vi>, error out=w484:errorcluster)
        n174 = Close Reference(reference=w483, error in (no error)=w484) -> (error out=w475:errorcluster)
        n175 = global read "AOI List Globals.vi" "AOI List"() -> (w482:u16[][])
        n176 = for {
          tunnel: w482 -> [w515] mode=indexing
          shift-right: [w518] -> w473
          shift-left: w475 -> [w520]
          shift-right: [w522] -> w466
          shift-left: w467 -> [w523]
          i -> [w521]
          w513 = u32 16711680 ("Color")
          n177 = call "AOI to optional rectangle.vi"("x1, y1, x2, y2 with origin (0, 0)"=w515) -> ("Rectangle Out"=w512:T13)  [unwired: 4 out]
          n178 = Unbundle By Name(w512) -> ("Left"=w510:i32, "Top"=w509:i32)
          n179 = Increment(x=w521) -> (x+1=w516:i32)
          n180 = call "IMAQ Overlay Rectangle"("Color"=w513, "error in (no error)"=w520, "Rectangle"=w512, "Image"=w523) -> ("error out"=w519:errorcluster, "Image Out"=w517:T9)  [unwired: 2 in, 4 out]
          n181 = Number To Decimal String(number=w516) -> (decimal integer string=w514:string)  [unwired: 1 out]
          n182 = Bundle("Left"=w510, "Top"=w509) -> (w511:cluster{"Left":i32, "Top":i32})  [unwired: 1 out]
          n183 = call "IMAQ Overlay Text"("Text Color (black)"=w513, "error in (no error)"=w519, "String"=w514, "Origin"=w511, "Image"=w517) -> ("error out"=w518:errorcluster, "Image Out"=w522:T9)  [unwired: 3 in, 2 out]
        }
      }
      event "Save Portion of Current Frame": Value Change {
        w530 = FALSE  # Redisplay image
        w531 = FALSE  # Reset control scales?
        n184 = event-data() -> ()  [unwired: 7 out]
        n185 = local read "Acquisition refnum array"() -> (w537:refnum<file>[])
        n186 = local read "Header data"() -> (w535:T2)
        n187 = call "GLIMPSE Save image.vi"("Header data"=w535, "Acqisition files refnums"=w537, "Frame number"=w533) -> ()  [unwired: 2 in, 6 out]
        n188 = local write "Tab Control"(enum32{"Controls", "FOV", "Tools", "Tracking"}."Controls" ("Tab Control")) -> ()
      }
      event "Print Image": Value Change {
        w552 = FALSE  # Redisplay image
        w553 = FALSE  # Reset control scales?
        w566 = "\r"
        # "4- print image"
        n189 = event-data() -> ()  [unwired: 7 out]
        n190 = local write "Tab Control"(enum32{"Controls", "FOV", "Tools", "Tracking"}."Controls" ("Tab Control")) -> ()
        n191 = global read "GLIMPSE Globals.vi" "Current window Black/White Levels"() -> (w569:cluster{ext, ext})
        n192 = property on="Printer" class="Ring (strict)"(error in=w551) -> (error out=w539:errorcluster, "Strings []"=w555:string[])  [unwired: 1 in, 1 out]
        n193 = local read "file path"() -> (w567:path)
        n194 = Unbundle(w569) -> (w560:ext, w561:ext)
        n195 = Number To Decimal String(number=w548) -> (decimal integer string=w558:string)  [unwired: 1 out]
        n196 = Index Array(array=w555, index="Printer") -> (element=w557:string)
        n197 = Path To String(path=w567) -> (string=w568:string)
        n198 = Number To Decimal String(number=w560) -> (decimal integer string=w564:string)  [unwired: 1 out]
        n199 = Number To Decimal String(number=w561) -> (decimal integer string=w562:string)  [unwired: 1 out]
        n200 = Concatenate Strings(w568, w566, "Black: " ("string"), w564, " White: " ("string"), w562, w566, "Frame " ("Printout title"), w558) -> (w542:string)
        n201 = case shown="1, Default" w543 {
          tunnel: w542 -> [w570 w574]
          tunnel: [w570 w575] -> w541
          tunnel: w540 -> [_ w571]
          frame 0 {
          }
          frame 1, Default {
            n202 = Number To Decimal String(number=w571) -> (decimal integer string=w572:string)  [unwired: 1 out]
            n203 = Concatenate Strings(w574, " of FOV " ("string"), w572) -> (w575:string)
          }
        }
        n204 = local read "Overlay?"() -> (w544:bool)
        n205 = call "Print AOI images.vi"("Black/White Levels"=w569, "AOI Overlay?"=w544, "error in (no error)"=w539, "printer name (default)"=w557, "Printout title"=w541, "Image In"=w550) -> ("error out"=w538:errorcluster)  [unwired: 4 out]
      }
      event "Save Sequence": Value Change {
        w585 = FALSE  # Redisplay image
        w586 = FALSE  # Reset control scales?
        n206 = event-data() -> ()  [unwired: 7 out]
        n207 = local read "Acquisition refnum array"() -> (w589:refnum<file>[])
        n208 = global read "GLIMPSE Globals.vi" "Current window Black/White Levels"() -> (w590:cluster{ext, ext})
        n209 = local read "Header data"() -> (w587:T2)
        n210 = local read "Frame Number"() -> (w588:cluster{u32, u32})
        n211 = global write "GLIMPSE Globals.vi" "Sequence range"(w588) -> ()
        n212 = local write "Tab Control"(enum32{"Controls", "FOV", "Tools", "Tracking"}."Controls" ("Tab Control")) -> ()
        n213 = call "GLIMPSE Sequence Save.vi"("Header file data"=w587, "Acquisition refnum array"=w589, "Black/White Levels"=w590) -> ()  [unwired: 1 in, 6 out]
      }
      event "FOV Mode", "Display FOV number", "Total FOVs": Value Change {
        n214 = event-data() -> ()  [unwired: 7 out]
        n215 = property on="Display FOV number" class="Slide (strict)"(error in=w594, "Scale.Maximum"="Total FOVs") -> (error out=w593:errorcluster)  [unwired: 1 in, 1 out]
        n216 = case shown="\"Display one field of view\"" "FOV Mode" {
          tunnel: [w611 i16 1 ("Display FOV number")] -> w604
          tunnel: [w610 i16 0 ("Total FOVs")] -> w605
          tunnel: w597 -> [w614 w615]
          tunnel: [w613 w615] -> w602
          tunnel: "Total FOVs" -> [w610 _]
          tunnel: "Display FOV number" -> [w609 _]
          frame "Display one field of view" {
            n217 = In Range and Coerce(upper limit=w610, x=w609, lower limit=i16 1) -> (coerced(x)=w611:i16)  [unwired: 1 out]
            n218 = Quotient & Remainder(x=w614, y=w610) -> (floor(x/y)=w613:u32)  [unwired: 1 out]
            n219 = local write "Display FOV number"(w611) -> ()
          }
          frame "Display all frames", Default {
          }
        }
        n220 = In Range and Coerce(upper limit=w602, x=w601, lower limit=u32 1) -> (coerced(x)=w598:u32)  [unwired: 1 out]
        n221 = local write "Current Frame Number"(w598) -> ()
      }
      event "Current Frame Number": Value Change {
        w626 = TRUE  # Redisplay image
        w627 = FALSE  # Reset control scales?
        n222 = event-data() -> ()  [unwired: 7 out]
      }
    }
    n223 = case shown="True" w58 {
      tunnel: w39 -> [_ w124]
      tunnel: w49 -> [w120 w126]
      tunnel: [w120 w125] -> w48
      frame False {
      }
      frame True {
        n224 = flat-sequence {
          tunnel: w126 -> [w131]
          tunnel: w124 -> [w127]
          tunnel: [w129] -> w123
          tunnel: [w128] -> w122
          tunnel: [w127] -> w121
          tunnel: [w139] -> w125
          tunnel: w123 -> [w139]
          tunnel: w122 -> [w134]
          tunnel: w121 -> [w133]
          frame #0 {
            w128 = u32 1
            n225 = property on="Current Frame Number" class="Slide (strict)"(error in=w131, "Scale.Range:Maximum"=w127, "Scale.Range:Minimum"=w128, "Maximum"=w127) -> (error out=w130:errorcluster)  [unwired: 1 in, 1 out]
            n226 = property on="Frame Number" class="Slide (strict)"(error in=w130, "Scale.Range:Maximum"=w127, "Scale.Range:Minimum"=w128, "Maximum"=w127) -> (error out=w129:errorcluster)  [unwired: 1 in, 1 out]
          }
          frame #1 {
            n227 = local read "Frame Number"() -> (w138:cluster{u32, u32})
            n228 = Unbundle(w138) -> (w135:u32, w136:u32)
            n229 = In Range and Coerce(upper limit=w133, x=w135, lower limit=w134) -> (coerced(x)=w132:u32)  [unwired: 1 out]
            n230 = Bundle("# of Frames in sequence"=w132, w136) -> (w137:cluster{"# of Frames in sequence":u32, u32})  [unwired: 1 out]
            n231 = local write "Frame Number"(w137) -> ()
          }
        }
      }
    }
    n232 = case shown="True" w50 {
      tunnel: w57 -> [w75 w111]
      tunnel: [errorcluster {"status"=FALSE, "code"=0, "source"=""} ("error out") w104] -> w43
      tunnel: [w75 w100] -> w56
      tunnel: w34 -> [_ w90]
      tunnel: w47 -> [_ w92]
      tunnel: w46 -> [_ w94]
      tunnel: w48 -> [_ w93]
      frame False {
        # "Don't display frame if we are about to quit."
      }
      frame True {
        # "Display frame"
        # "Display current frame"
        n233 = local read "Header2 data"() -> (w89:T1)
        n234 = Decrement(x=w90) -> (x-1=w91:u32)
        n235 = local write "Current Frame Number"(w90) -> ()
        n236 = local read "Header data"() -> (w105:T2)
        n237 = local read "Acquisition refnum array"() -> (w109:refnum<file>[])
        n238 = call "GLIMPSE Fetch Image.vi"("Display FOV number"=w94, "Total FOVs"=w92, "Header file data"=w105, "Acqisition files refnums"=w109, "error in"=w93, "Logical Frame Number\n(starting with zero)"=w91, "Image In"=w111) -> ("error out"=w97:errorcluster, "Image Out"=w99:T9)  [unwired: 2 in, 1 out]
        n239 = Unbundle By Name(w89) -> ("Lasers array"=w88:u16[][], "Filter array"=w86:u16[], "Flow rate array"=w82:dbl[], "Temperature array"=w84:dbl[], "Field array"=w83:u16[])
        n240 = Unbundle By Name(w105) -> ("TTB Array (ms)"=w106:u32[], "Element 0 of TTB"=w107:u32, "Pixel depth"=w102:u32)
        n241 = call "GLIMPSE fetch TTB value.vi"("Array of TTB Values (ms)"=w106, "Logical Frame Number\n(starting with zero)"=w91) -> ("Array index"=w81:u32, "TTB value out"=w108:u32)  [unwired: 5 out]
        "Time\nStamp" <- w108
        n242 = call "Add AOIs overlay to image.vi"("error in (no error)"=w97, "Current frame number\n(starting with 1)"=w90, "Overlay on?"="Overlay?", "Image Src"=w99) -> ("error out"=w96:errorcluster, "Image Dst"=w98:T9)  [unwired: 2 in, 4 out]
        n243 = Index Array(array=w83, index=w81) -> (element=→"Field":u16)
        n244 = Subtract(x=w108, y=w107) -> (x-y=→"Time after 1st\nFrame (ms)":u32)
        n245 = Index Array(array=w84, index=w81) -> (element=→"Temp":dbl)
        n246 = Index Array(array=w86, index=w81) -> (element=→"Filter":u16)
        n247 = Index Array(array=w88, index (row)=w81) -> (element=w87:u16[])  [unwired: 1 in]
        n248 = Index Array(array=w82, index=w81) -> (element=→"Flow":dbl)
        n249 = for {
          N: "# Display\nWindows" -> [_]
          tunnel: w98 -> [w119]
          tunnel: [w118] -> w100
          tunnel: [w117] -> w104
          tunnel: w96 -> [w116]
          tunnel: "Seq. Player" ("Title") -> [w115]
          tunnel: w102 -> [w114]
          i -> [w112]
          n250 = call "Send image to image display controller.vi"("Image"=w119, "Window Title"=w115, "Window Number"=w112, "error in"=w116, "Image Type"=w114, "Quit display controller?"=FALSE) -> ("Image Out"=w118:T9, "error out"=w117:errorcluster)  [unwired: 1 in, 2 out]
        }
        n251 = Not Equal To 0?(x=w87) -> (x != 0?=→"Lasers":bool[])
      }
    }
    n252 = case shown="\"Play Backward\"" w38 {
      tunnel: [TRUE w72 w73] -> w53
      tunnel: [w69 w72 TRUE] -> w52
      tunnel: [w69 TRUE w73] -> w51
      frame "Stop", Default {
        w69 = FALSE
      }
      frame "Play Forward" {
        w72 = FALSE
      }
      frame "Play Backward" {
        w73 = FALSE
      }
    }
    n253 = Unbundle By Name(w43) -> ("status"=w54:bool)
    n254 = Or(x=w54, y="Exit") -> (x .or. y?=w44:bool)
    n255 = property on="Fwd bkd" class="Bool (strict)"("Visible"=w51) -> ()  [unwired: 2 in, 2 out]
    n256 = property on="Stop bkgd" class="Bool (strict)"("Visible"=w53) -> ()  [unwired: 2 in, 2 out]
    n257 = property on="Rev bkd" class="Bool (strict)"("Visible"=w52) -> ()  [unwired: 2 in, 2 out]
  }
  n258 = stacked-sequence {
    tunnel: w12 -> [w633]
    tunnel: w2 -> [w630]
    tunnel: [w629] -> w1
    frame #0 {
      # "Shutdown"
      n259 = call "IMAQ Dispose"("error in (no error)"=w630) -> ("error out"=w636:errorcluster)  [unwired: 2 in, 3 out]
      n260 = local read "Frame Number"() -> (w634:cluster{u32, u32})
      "Sequence Range" <- w634
      n261 = call "Open caller's caller.vi"("vi reference"=w633) -> ()  [unwired: 1 in, 7 out]
      n262 = call "IMAQ WindToolsClose"("error in (no error)"=w636) -> ("error out"=w631:errorcluster)  [unwired: 5 out]
      n263 = call "Send image to image display controller.vi"("error in"=w631, "Quit display controller?"=TRUE) -> ("error out"=w629:errorcluster)  [unwired: 5 in, 3 out]
      n264 = global write "GLIMPSE Globals.vi" "Sequence range"(w634) -> ()
      n265 = local read "Acquisition refnum array"() -> (w635:refnum<file>[])
      n266 = for {
        tunnel: w635 -> [w637] mode=indexing
        n267 = Close File(refnum=w637) -> ()  [unwired: 1 in, 2 out]
      }
    }
  }
  n268 = call "Glimpse error handler.vi"("error in"=w1) -> ()  [unwired: 1 in, 6 out]
